vi "RemoteVI Hover Menus.vi"(0 "hWnd":u64, 5 "state":T1, 7 "now":u32) -> (4 "state out":T1)   [LabVIEW 2020, in "RemoteVI.lvlib"]
doc: "One hover step of RemoteVI Menu Hover.vi: lists the open LabVIEW menus (RemoteVI List Menus.vi), decides what the remote pointer asks of them (RemoteVI Hover Decision.vi) and does it with keys - over the deepest menu the highlight follows the pointer (RemoteVI Hover Navigate.vi); after 400 ms on one item VK_RIGHT opens its submenu (RemoteVI Post Menu Key.vi; dwelled is set, so it is decided once) - but only when that item shows a submenu arrow (RemoteVI Menu Highlight.vi submenu?), because in a menu of the panel's menu bar VK_RIGHT on an item without a submenu opens the next menu bar menu (measured); over a parent of open submenus RemoteVI Hover Parent Menu.vi. state out is the updated menu pointer state; the caller stores it. Errors are dropped. No VI Server call."
uses:
  RemoteVI.lvlib
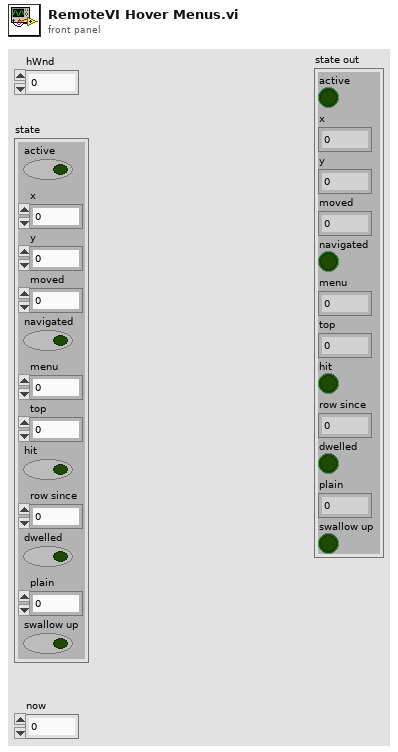
[diagram p1: front panel]
types:
  T1 = cluster{"active":bool, "x":i32, "y":i32, "moved":u32, "navigated":bool, "menu":u64, "top":i32, "hit":bool, "row since":u32, "dwelled":bool, "plain":u64, "swallow up":bool}
  T2 = cluster{"hwnd":u64, "x":i32, "y":i32, "w":i32, "h":i32}[]
  T3 = cluster{"hwnd":u64, "x":i32, "y":i32, "w":i32, "h":i32}
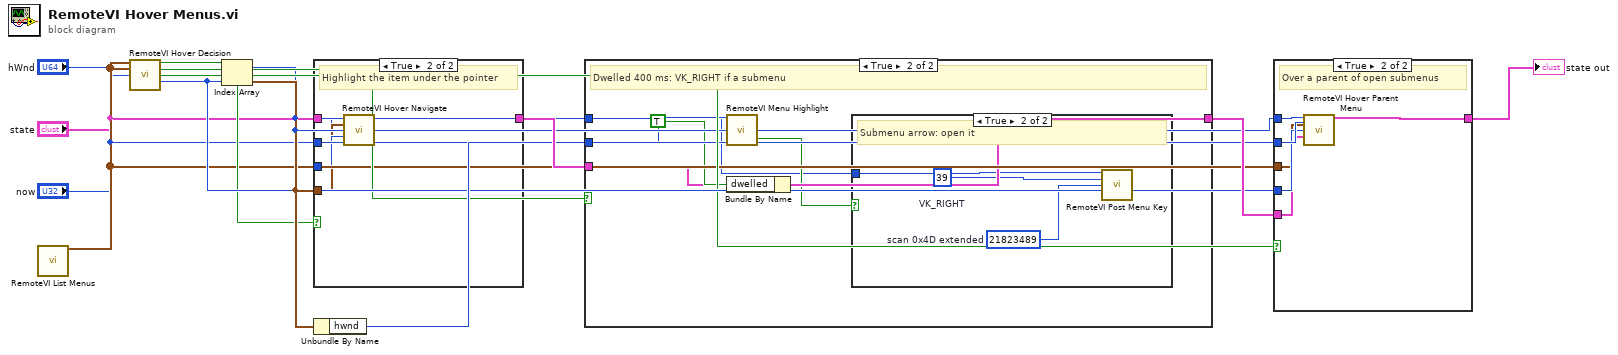
[diagram p0: block diagram]
diagram:
  n1 = call "RemoteVI List Menus.vi"() -> ("menus"=w4:T2)  [unwired: 15 in]
  n2 = call "RemoteVI Hover Decision.vi"("menus"=w4, "state"="state", "now"="now") -> ("navigate?"=w5:bool, "dwell?"=w6:bool, "parent?"=w7:bool, "k"=w8:i32)  [unwired: 9 in]
  n3 = Index Array(array=w4, index=w8) -> (element=w9:T3)
  n4 = case shown="True" w5 {
    tunnel: "state" -> [w14 w15]
    tunnel: "hWnd" -> [_ w16]
    tunnel: "now" -> [_ w18]
    tunnel: w9 -> [_ w17]
    tunnel: [w14 w19] -> w11
    frame False {
    }
    frame True {
      # "Highlight the item under the pointer"
      n5 = call "RemoteVI Hover Navigate.vi"("hWnd"=w16, "menu"=w17, "state"=w15, "now"=w18) -> ("state out"=w19:T1)  [unwired: 10 in, 1 out]
    }
  }
  n6 = Unbundle By Name(w9) -> ("hwnd"=w10:u64)
  n7 = case shown="True" w6 {
    tunnel: "hWnd" -> [_ w22]
    tunnel: w10 -> [_ w23]
    tunnel: w11 -> [w20 w21]
    tunnel: [w20 w26] -> w12
    frame False {
    }
    frame True {
      # "Dwelled 400 ms: VK_RIGHT if a submenu"
      n8 = call "RemoteVI Menu Highlight.vi"("hwnd"=w23) -> ("submenu?"=w24:bool)  [unwired: 8 in, 6 out]
      n9 = Bundle By Name(cluster=w21, "dwelled"=TRUE) -> (w26:T1)
      n10 = case shown="True" w24 {
        tunnel: w22 -> [_ w27]
        frame False {
        }
        frame True {
          w29 = i64 21823489  # scan 0x4D extended
          w28 = u64 39  # VK_RIGHT
          # "Submenu arrow: open it"
          n11 = call "RemoteVI Post Menu Key.vi"("hWnd"=w27, "vk"=w28, "key lParam"=w29) -> ()  [unwired: 12 in, 1 out]
        }
      }
    }
  }
  n12 = case shown="True" w7 {
    tunnel: "hWnd" -> [_ w32]
    tunnel: "now" -> [_ w35]
    tunnel: w4 -> [_ w33]
    tunnel: w8 -> [_ w34]
    tunnel: w12 -> [w30 w31]
    tunnel: [w30 w36] -> w13
    frame False {
    }
    frame True {
      # "Over a parent of open submenus"
      n13 = call "RemoteVI Hover Parent Menu.vi"("hWnd"=w32, "now"=w35, "menus"=w33, "k"=w34, "state"=w31) -> ("state out"=w36:T1)  [unwired: 9 in, 1 out]
    }
  }
  "state out" <- w13
